vi "input.vi"(8 "error in":errorcluster, 10 "data table in":T1, 11 "J1939 runtime in":refnum<class "J1939 runtime.lvclass">) -> (0 "error out":errorcluster, 2 "data table out":T1, 3 "J1939 runtime out":refnum<class "J1939 runtime.lvclass">)   [LabVIEW 2015, in "J1939 runtime.lvclass"]
doc: "Provides an interface for reading data from a module at runtime. While this interface performs no operations, a child should provide an override which may read from any open sessions, references, or interfaces."
uses:
  J1939 runtime.lvclass
  <vilib>/NI/Tag Bus/table/data table.ctl
  <vilib>/xnet/xnet.llb/XNET CAN Comm State.ctl
  J1939 runtime.lvclass/J1939 runtime.ctl
  <vilib>/xnet/xnet.llb/XNET Control Scope.ctl
  <vilib>/xnet/xnet.llb/XNET Read (Signal Single-point).vi
  <vilib>/xnet/xnet.llb/XNET Read (State CAN Comm).vi
  <vilib>/NI/Tag Bus/table/data table.lvlib
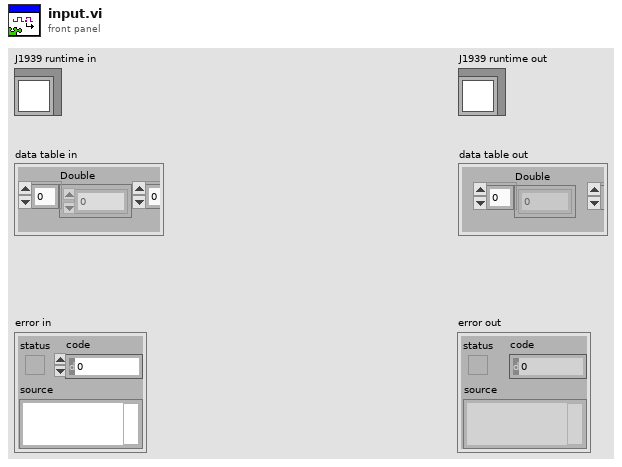
[diagram p1: front panel]
types:
  T1 = typedef "tag bus.lvlib/data table.lvlib/data table.ctl" = cluster{"Double":dbl[], "Single":sgl[], "I64":i64[], "I32":i32[], "I16":i16[], "I8":i8[], "U64":u64[], "U32":u32[], "U16":u16[], "U8":u8[], "Boolean":bool[], "String":string[], "Array of Double":cluster{"DBL Array":dbl[]}[], "Array of Single":cluster{"SGL Array":sgl[]}[], "Array of I64":cluster{"I64 Array":i64[]}[], "Array of I32":cluster{"I32 Array":i32[]}[], "Array of I16":cluster{"I16 Array":i16[]}[], "Array of I8":cluster{"I8 Array":i8[]}[], "Array of U64":cluster{"U64 Array":u64[]}[], "Array of U32":cluster{"U32 Array":u32[]}[], "Array of U16":cluster{"U16 Array":u16[]}[], "Array of U8":cluster{"U8 Array":u8[]}[], "Array of Boolean":cluster{"Boolean Array":bool[]}[], "Array of String":cluster{"String Array":string[]}[]}
  T2 = typedef "XNET CAN Comm State.ctl" = u8
  T3 = typedef "J1939 configuration.lvclass/Signal Mapping.ctl" = cluster{"data type":T4, "index":i32}
  T4 = typedef "tag bus.lvlib/tag descriptor.lvclass/Data Type.ctl" = enum16{"Double", "Single", "I64", "I32", "I16", "I8", "U64", "U32", "U16", "U8", "Boolean", "String", "Array of Double", "Array of Single", "Array of I64", "Array of I32", "Array of I16", "Array of I8", "Array of U64", "Array of U32", "Array of U16", "Array of U8", "Array of Boolean", "Array of String"}
  T5 = typedef "XNET CAN Comm.ctl" = cluster{"fault code":i32, "fault?":bool, "communication state":T2, "last error":T6, "receive error counter":u8, "transmit error counter":u8, "transceiver error?":bool, "sleep?":bool}
  T6 = typedef "XNET CAN Last Err.ctl" = u8
  T7 = typedef "XNET Control Scope.ctl" = u32
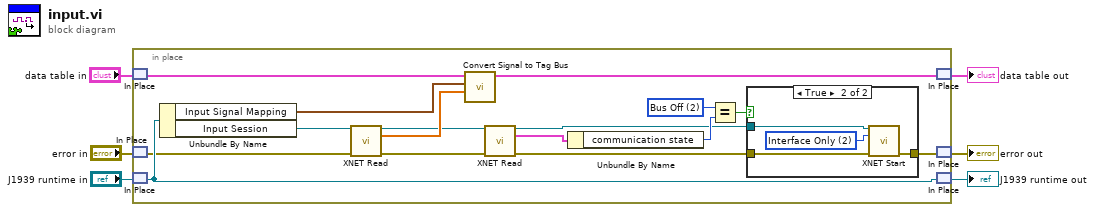
[diagram p0: block diagram]
diagram:
  n1 = in-place {
    w12 = T2 2 items=["Error Active", "Error Passive", "Bus Off", "Init"] ("x")
    n2 = in-place-match #1("data table in") -> (w21:T1)
    n3 = in-place-match #2("error in") -> (w17:errorcluster)
    n4 = in-place-match #3("J1939 runtime in") -> (w22:refnum<class "J1939 runtime.lvclass">)
    n5 = Unbundle By Name(w22) -> ("Input Signal Mapping"=w19:T3[], "Input Session"=w7:refnum<k21>)
    n6 = call-poly <vilib>:"XNET Read.vi"("session in"=w7, "error in (no error)"=w17) -> ("session out"=w16:refnum<k21>, "data"=w18:dbl[], "error out"=w15:errorcluster)  [unwired: 11 out]
    n7 = call "Convert Signal to Tag Bus.vi"("Signals"=w18, "signal mapping"=w19, "data table in in"=w21) -> ("data table out 2"=w20:T1)  [unwired: 8 in]
    n8 = call-poly <vilib>:"XNET Read.vi"("session in"=w16, "error in (no error)"=w15) -> ("session out"=w10:refnum<k21>, "CAN comm"=w14:T5, "error out"=w9:errorcluster)  [unwired: 11 in]
    n9 = Unbundle By Name(w14) -> ("communication state"=w13:T2)
    n10 = Equal?(x=w12, y=w13) -> (x = y?=w11:bool)
    n11 = case shown="True" w11 {
      tunnel: w10 -> [_ w27]
      tunnel: w9 -> [w23 w25]
      tunnel: [w23 w24] -> w8
      frame False {
      }
      frame True {
        w26 = T7 2 items=["Normal", "Session Only", "Interface Only", "Session Only Blocking"] ("scope (normal)")
        n12 = call <vilib>:"XNET Start.vi"("session in"=w27, "scope (normal)"=w26, "error in (no error)"=w25) -> ("error out"=w24:errorcluster)  [unwired: 11 in, 1 out]
      }
    }
    n13 = in-place-match #1(w20) -> (→"data table out":T1)
    n14 = in-place-match #2(w8) -> (→"error out":errorcluster)
    n15 = in-place-match #3(w22) -> (→"J1939 runtime out":refnum<class "J1939 runtime.lvclass">)
  }
